vi "Get Wf Time Information.vi"(11 "signal in":waveform(dbl)) -> (1 "dt":dbl, 2 "Final Time":timestamp, 3 "Start Time":timestamp)   [LabVIEW 2020, in "Data Viewer.lvlib" / "Data Viewer.lvclass"]
uses:
  Data Viewer.lvclass
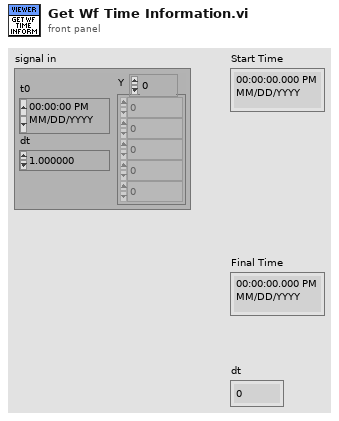
[diagram p1: front panel]
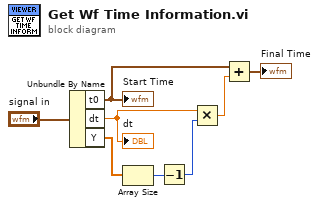
[diagram p0: block diagram]
diagram:
  n1 = Unbundle By Name("signal in") -> ("t0"=w6:timestamp, "dt"=w5:dbl, "Y"=w1:dbl[])
  "Start Time" <- w6
  "dt" <- w5
  n2 = Array Size(array=w1) -> (size(s)=w2:i32)
  n3 = Decrement(x=w2) -> (x-1=w8:i32)
  n4 = Multiply(x=w5, y=w8) -> (x*y=w3:dbl)
  n5 = Add(x=w6, y=w3) -> (x+y=→"Final Time":timestamp)
